vi "UI - Read IO Variables.vi"(0 "IO References":T1, 5 "Control Output Values":dbl[](array[numeric]), 7 "Array":bool[](array[boolean]), 9 "Control Output Values 2":dbl[](array[numeric]), 11 "error in (no error)":errorcluster, 12 "Array 2":bool[](array[boolean])) -> (4 "Control Input Values crio1":dbl[](array[numeric]), 10 "Input Values Crio2":dbl[](array[numeric]), 14 "Threshold Exceeded?":bool, 15 "error out":errorcluster)   [LabVIEW 2025]
uses:
  controls/IO References.ctl
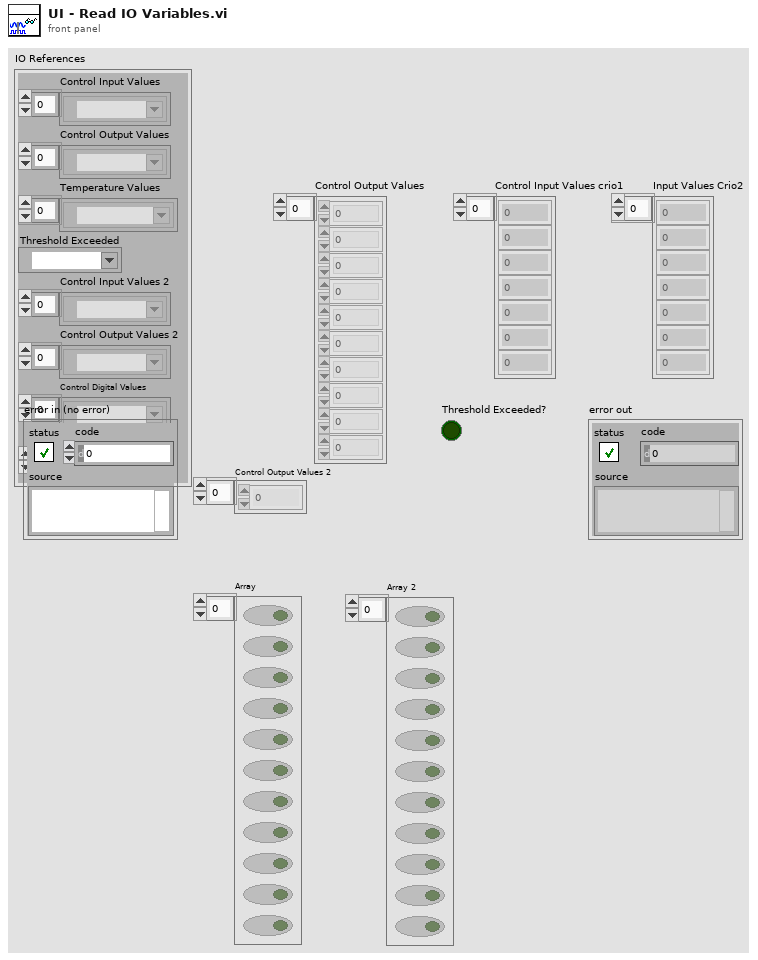
[diagram p1: front panel]
types:
  T1 = typedef "IO References.ctl" = cluster{"Control Input Values":refnum<k21>[], "Control Output Values":refnum<k21>[], "Temperature Values":refnum<k21>[], "Threshold Exceeded":refnum<k21>, "Control Input Values 2":refnum<k21>[], "Control Output Values 2":refnum<k21>[], "Control Digital Values":refnum<k21>[], "Control Digital Values 2":refnum<k21>[]}
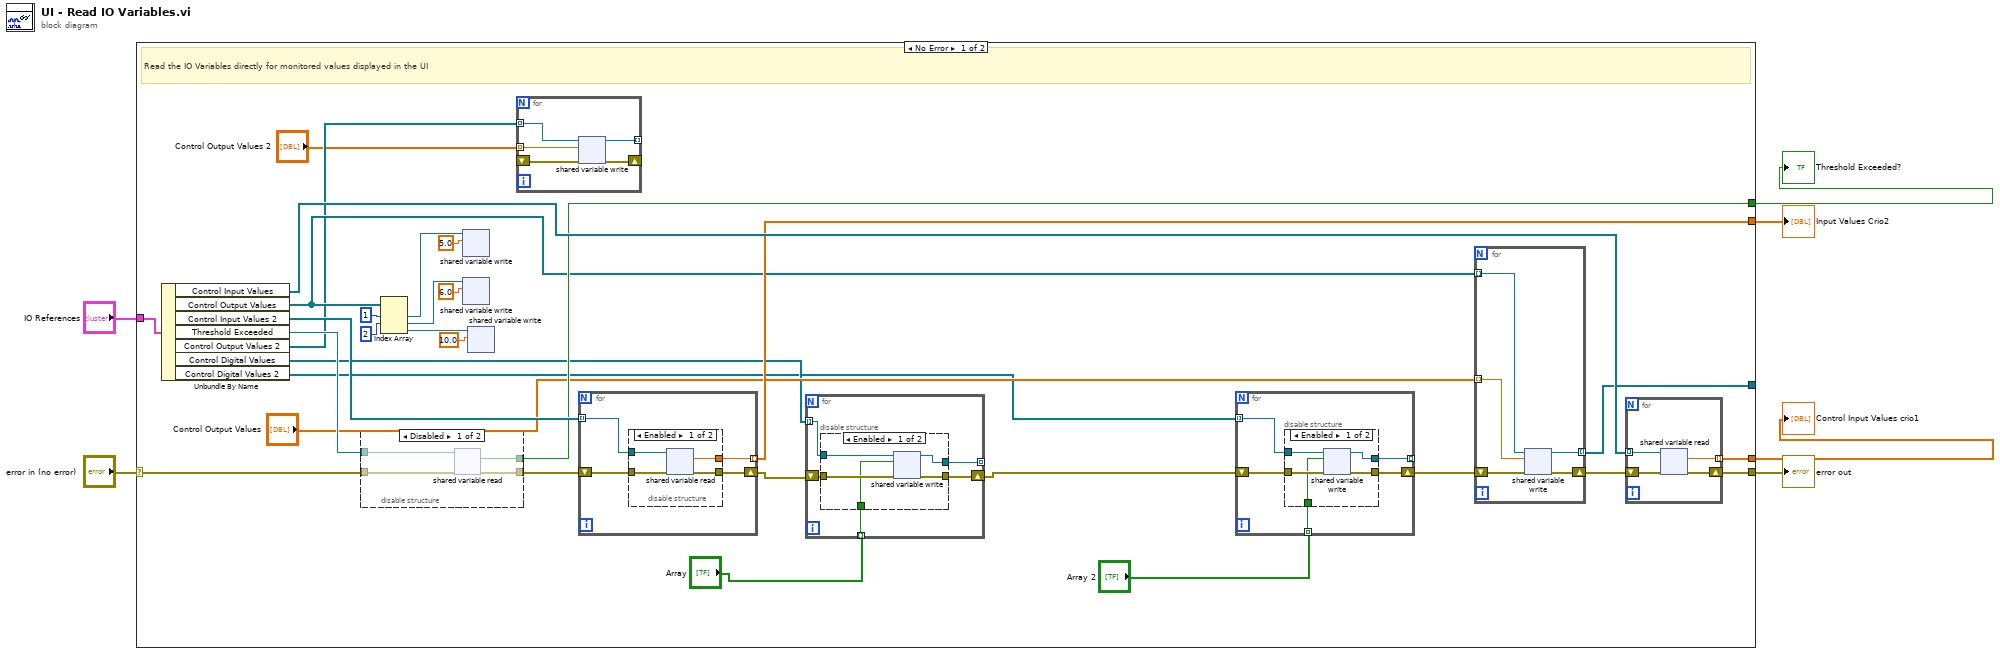
[diagram p0: block diagram]
diagram:
  n1 = case shown="No Error" "error in (no error)" {
    selector: "error in (no error)" -> [w26 w88]
    tunnel: "IO References" -> [w37 _]
    tunnel: [w31 w88] -> w5
    tunnel: [w30 _] -> w4
    tunnel: [w29 _] -> w3
    tunnel: [w28 _] -> _
    tunnel: [w27 _] -> w2
    frame No Error {
      # "Read the IO Variables directly for monitored values displayed in the UI"
      n2 = Unbundle By Name(w37) -> ("Control Input Values"=w32:refnum<k21>[], "Control Output Values"=w25:refnum<k21>[], "Control Input Values 2"=w34:refnum<k21>[], "Threshold Exceeded"=w36:refnum<k21>, "Control Output Values 2"=w15:refnum<k21>[], "Control Digital Values"=w13:refnum<k21>[], "Control Digital Values 2"=w11:refnum<k21>[])
      n3 = disable-structure shown="Disabled" {
        disable-tunnel: w36 -> [w68 _]
        disable-tunnel: [w67 w69] -> w35
        disable-tunnel: [w66 _] -> w30
        disable-tunnel: w26 -> [w65 w69]
        frame Disabled {
          n4 = shared-variable-read(w68, w65) -> (w67:errorcluster, w66:bool)  [unwired: 2 out]
        }
        frame Enabled {
        }
      }
      n5 = Index Array(array=w25, index #1=1 ("index"), index #2=2 ("index")) -> (element #1=w23:refnum<k21>, element #2=w20:refnum<k21>, element #3=w18:refnum<k21>)  [unwired: 1 in]
      n6 = shared-variable-write(w23, 5.0 ("data in")) -> ()  [unwired: 1 in, 2 out]
      n7 = shared-variable-write(w20, 6.0 ("data in")) -> ()  [unwired: 1 in, 2 out]
      n8 = shared-variable-write(w18, 10.0 ("data in")) -> ()  [unwired: 1 in, 2 out]
      n9 = for {
        shift-right: [w63] -> _
        shift-left: _ -> [w64]
        tunnel: [w62] -> _ mode=indexing
        tunnel: "Control Output Values 2" -> [w61] mode=indexing
        tunnel: w15 -> [w60] mode=indexing
        n10 = shared-variable-write(w60, w64, w61) -> (w62:refnum<k21>, w63:errorcluster)
      }
      n11 = for {
        shift-right: [w80] -> w12
        shift-left: w35 -> [w81]
        tunnel: w34 -> [w82] mode=indexing
        tunnel: [w79] -> w29 mode=indexing
        n12 = disable-structure shown="Enabled" {
          disable-tunnel: w82 -> [w86 _]
          disable-tunnel: w81 -> [w85 w87]
          disable-tunnel: [w84 w87] -> w80
          disable-tunnel: [w83 _] -> w79
          frame Enabled {
            n13 = shared-variable-read(w86, w85) -> (w84:errorcluster, w83:dbl)  [unwired: 2 out]
          }
          frame Disabled {
          }
        }
      }
      n14 = for {
        shift-right: [w51] -> w7
        shift-left: w12 -> [w52]
        tunnel: w13 -> [w53] mode=indexing
        tunnel: [w50] -> _ mode=indexing
        tunnel: "Array" -> [w49] mode=indexing
        n15 = disable-structure shown="Enabled" {
          disable-tunnel: w53 -> [w58 _]
          disable-tunnel: w52 -> [w57 w59]
          disable-tunnel: [w56 w59] -> w51
          disable-tunnel: [w55 _] -> w50
          disable-tunnel: w49 -> [w54 _]
          frame Enabled {
            n16 = shared-variable-write(w58, w57, w54) -> (w55:refnum<k21>, w56:errorcluster)
          }
          frame Disabled {
          }
        }
      }
      n17 = for {
        shift-right: [w40] -> w10
        shift-left: w7 -> [w41]
        tunnel: w11 -> [w42] mode=indexing
        tunnel: [w39] -> _ mode=indexing
        tunnel: "Array 2" -> [w38] mode=indexing
        n18 = disable-structure shown="Enabled" {
          disable-tunnel: w42 -> [w47 _]
          disable-tunnel: w41 -> [w46 w48]
          disable-tunnel: [w45 w48] -> w40
          disable-tunnel: [w44 _] -> w39
          disable-tunnel: w38 -> [w43 _]
          frame Enabled {
            n19 = shared-variable-write(w47, w46, w43) -> (w44:refnum<k21>, w45:errorcluster)
          }
          frame Disabled {
          }
        }
      }
      n20 = for {
        shift-right: [w76] -> w33
        shift-left: w10 -> [w77]
        tunnel: w25 -> [w78] mode=indexing
        tunnel: [w75] -> w28 mode=indexing
        tunnel: "Control Output Values" -> [w74] mode=indexing
        n21 = shared-variable-write(w78, w77, w74) -> (w75:refnum<k21>, w76:errorcluster)
      }
      n22 = for {
        shift-right: [w71] -> w31
        shift-left: w33 -> [w72]
        tunnel: w32 -> [w73] mode=indexing
        tunnel: [w70] -> w27 mode=indexing
        n23 = shared-variable-read(w73, w72) -> (w71:errorcluster, w70:dbl)  [unwired: 2 out]
      }
    }
    frame Error {
      # "Error"
    }
  }
  "error out" <- w5
  "Control Input Values crio1" <- w2
  "Input Values Crio2" <- w3
  "Threshold Exceeded?" <- w4
